vi "打开引用CSM.vi"(6 "子程序？":bool, 7 "引用":refnum<vi>, 8 "错误输入":errorcluster caption="错误输入（无错误）", 9 "CSM Name":string, 10 "VI":refnum<vi>) -> (0 "错误输出":errorcluster, 3 "VI输出":refnum<vi>)   [LabVIEW 2017]
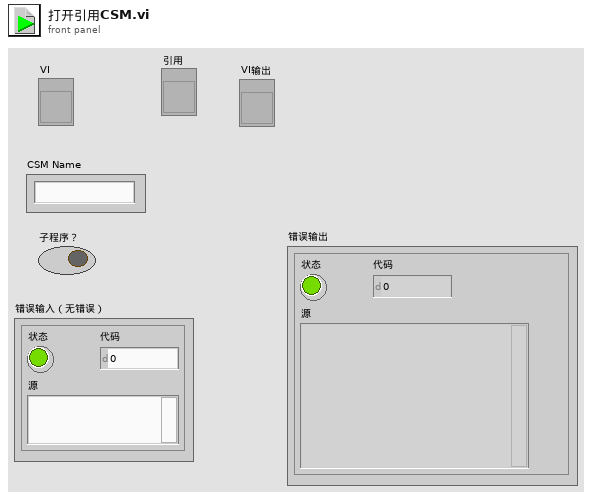
[diagram p1: front panel]
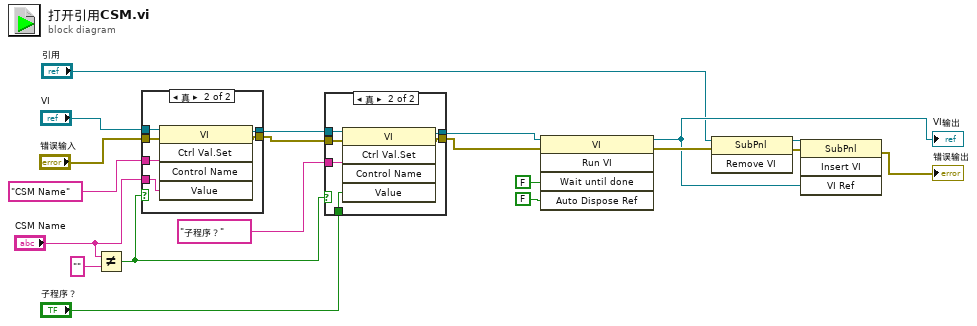
[diagram p0: block diagram]
diagram:
  n1 = Not Equal?(x="CSM Name", y="") -> (x != y?=w2:bool)
  n2 = case shown="真" w2 {
    tunnel: "VI" -> [w22 w28]
    tunnel: [w22 w27] -> w7
    tunnel: "CSM Name" ("控件名") -> [_ w26]
    tunnel: "CSM Name" -> [_ w25]
    tunnel: "错误输入" -> [w21 w24]
    tunnel: [w21 w23] -> w5
    frame False {
    }
    frame True {
      n3 = invoke class="VI" method="Ctrl Val.Set"(reference=w28, error in=w24, "Control Name"=w26, "Value"=w25) -> (reference out=w27:refnum<vi>, error out=w23:errorcluster)  [unwired: 1 in, 3 out]
    }
  }
  n4 = case shown="真" w2 {
    tunnel: w7 -> [w30 w36]
    tunnel: [w30 w35] -> w6
    tunnel: "子程序？" ("控件名") -> [_ w34]
    tunnel: w5 -> [w29 w33]
    tunnel: [w29 w32] -> w4
    tunnel: "子程序？" -> [_ w31]
    frame False {
    }
    frame True {
      n5 = invoke class="VI" method="Ctrl Val.Set"(reference=w36, error in=w33, "Control Name"=w34, "Value"=w31) -> (reference out=w35:refnum<vi>, error out=w32:errorcluster)  [unwired: 1 in, 3 out]
    }
  }
  n6 = invoke on="Invoke Node" class="VI" method="Run VI"(reference=w6, error in=w4, "Wait until done"=FALSE ("Wait Until Done"), "Auto Dispose Ref"=FALSE ("Auto Dispose Reference")) -> (reference out=w17:refnum<vi>, error out=w18:errorcluster)  [unwired: 1 in, 3 out]
  "VI输出" <- w17
  n7 = invoke class="SubPnl" method="Remove VI"(reference="引用", error in=w18) -> (reference out=w19:refnum<vi>, error out=w20:errorcluster)  [unwired: 1 in, 1 out]
  n8 = invoke class="SubPnl" method="Insert VI"(reference=w19, error in=w20, "VI Ref"=w17) -> (error out=→"错误输出":errorcluster)  [unwired: 1 in, 3 out]
